vi "Set Turn Table Speed.vi"(8 "error in (no error)":errorcluster, 11 "Interface - Turn Table in":refnum<class "Interface - Turn Table.lvclass">) -> (0 "error out":errorcluster, 3 "Interface - Turn Table out":refnum<class "Interface - Turn Table.lvclass">)   [LabVIEW 2023, in "Turn Table and Mast.lvlib" / "Interface - Turn Table.lvclass"]
uses:
  Interface - Turn Table.lvclass
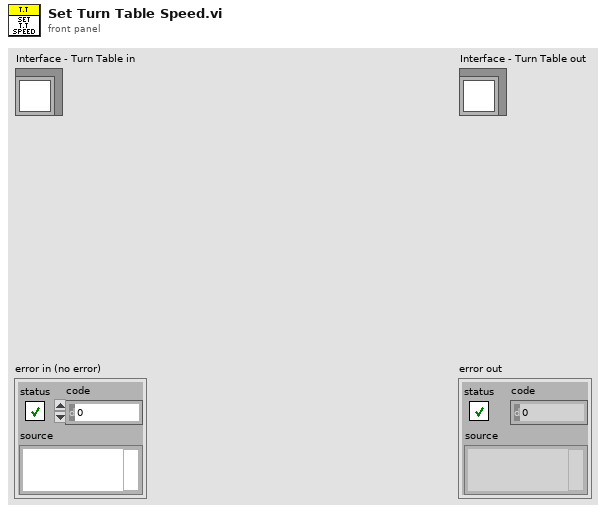
[diagram p1: front panel]
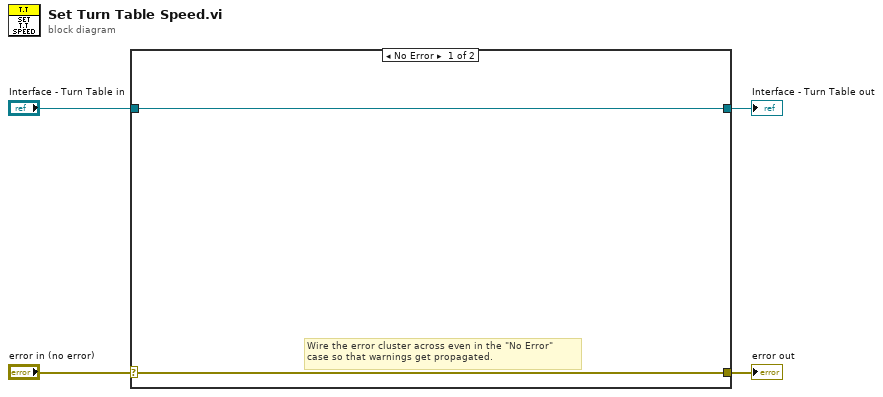
[diagram p0: block diagram]
diagram:
  n1 = case shown="No Error" "error in (no error)" {
    selector: "error in (no error)" -> [w5 w8]
    tunnel: [w5 w8] -> w3
    tunnel: [w6 w7] -> w1
    tunnel: "Interface - Turn Table in" -> [w6 w7]
    frame No Error {
      # "Wire the error cluster across even in the \"No Error\"\ncase so that warnings get propagated."
    }
    frame Error {
    }
  }
  "error out" <- w3
  "Interface - Turn Table out" <- w1
